vi "VIH UI - Append Control Rules - Ask If Add Duplicates.vi"(10 "Ctrl Rules (new)":T1[](array[typedef]), 11 "Ctrl Rules (existing)":T1[](array[typedef])) -> (2 "Ctrl Rules (new) out":T1[](array[typedef]))   [LabVIEW 2014]
doc: "::: VI Helpeks :::\nCopyright (c) 2000-2026 Konstantin Shifershteyn. All rights reserved."
uses:
  _VIH HelpGen.llb/VIH HelpGen Typedef - Cluster - Control Rule.ctl
  _VIH HelpGen.llb/VIH HelpGen Typedef - Enum - Description Mode.ctl
  _VIH HelpGen.llb/VIH HelpGen Typedef - Enum - Default,Enable,Disable.ctl
  _VIH HelpGen.llb/VIH HelpGen Typedef - Cluster - Enum Value Info.ctl
panel:
  # "VI Helpeks\nCopyright (c) 2012-2026 Konstantin Shifershteyn"
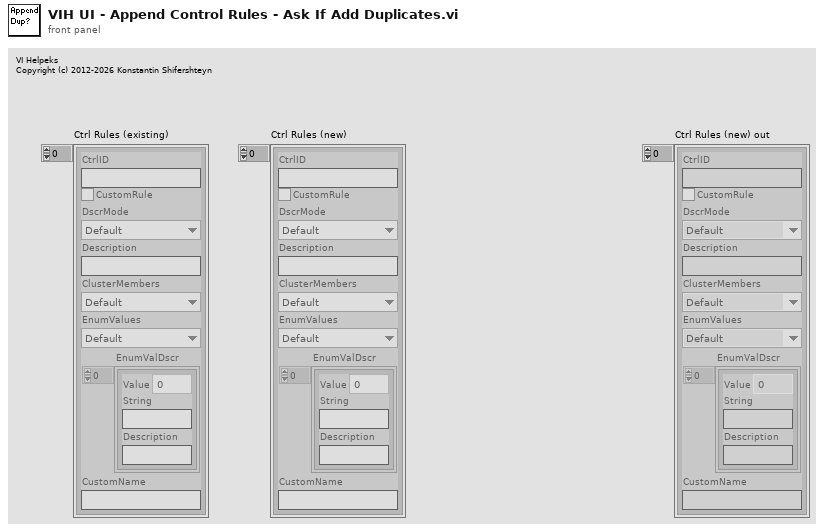
[diagram p1: front panel]
types:
  T1 = typedef "VIH HelpGen Typedef - Cluster - Control Rule.ctl" = cluster{"CtrlID":string, "CustomRule":bool, "DscrMode":T2, "Description":string, "ClusterMembers":T3, "EnumValues":T3, "EnumValDscr":T4[], "CustomName":string}
  T2 = typedef "VIH HelpGen Typedef - Enum - Description Mode.ctl" = enum16{"Default", "Description", "Description1", "Description2", "Custom", "None"}
  T3 = typedef "VIH HelpGen Typedef - Enum - Default,Enable,Disable.ctl" = enum16{"Default", "Enable", "Disable"}
  T4 = typedef "VIH HelpGen Typedef - Cluster - Enum Value Info.ctl" = cluster{"Value":ext, "String":string, "Description":string}
  T5 = enum16{"Left Button", "Center Button", "Right Button", "Window Close"}
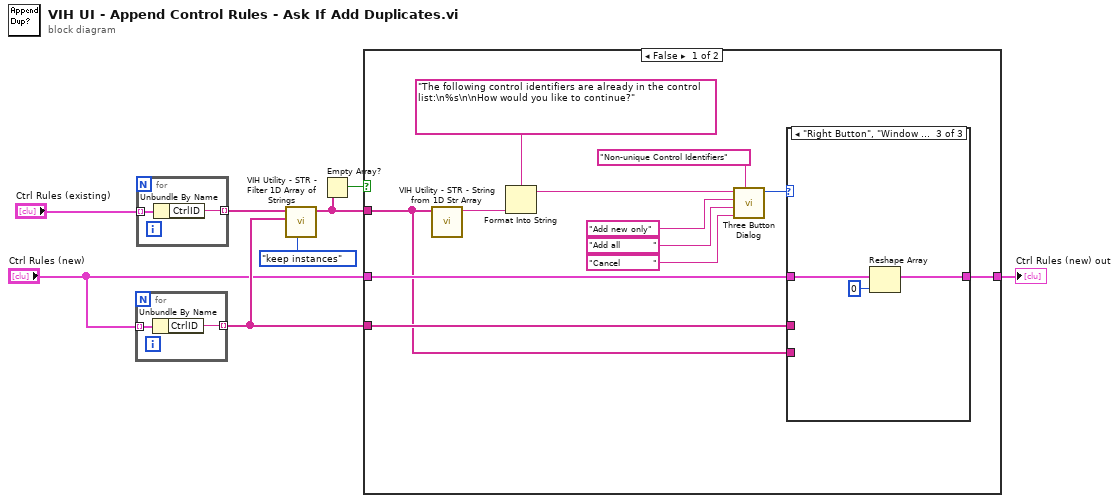
[diagram p0: block diagram]
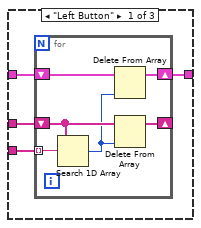
[diagram p2: hidden frame]
diagram:
  n1 = for {
    tunnel: "Ctrl Rules (new)" -> [w10] mode=indexing
    tunnel: [w9] -> w3 mode=indexing
    n2 = Unbundle By Name(w10) -> ("CtrlID"=w9:string)
  }
  n3 = for {
    tunnel: "Ctrl Rules (existing)" -> [w12] mode=indexing
    tunnel: [w11] -> w7 mode=indexing
    n4 = Unbundle By Name(w12) -> ("CtrlID"=w11:string)
  }
  n5 = call "VIH Utility - STR - Filter 1D Array of Strings.vi"("Action (keep instances)"=enum16{"keep instances", "remove instances"}."keep instances", "instances"=w3, "Array in"=w7) -> ("Array out"=w4:string[])  [unwired: 7 in, 1 out]
  n6 = Empty Array?(array=w4) -> (empty?=w5:bool)
  n7 = case shown="False" w5 {
    tunnel: w4 -> [w21 _]
    tunnel: w3 -> [w24 _]
    tunnel: "Ctrl Rules (new)" -> [w23 w39]
    tunnel: [w22 w39] -> w1
    frame False {
      n8 = call "VIH Utility - STR - String from 1D Str Array.vi"("Array in"=w21) -> ("String out"=w20:string)  [unwired: 6 in]
      n9 = Format Into String(format string="The following control identifiers are already in the control list:\n%s\n\nHow would you like to continue?", w20) -> (resulting string=w18:string)  [unwired: 2 in, 1 out]
      n10 = call <vilib>:"Three Button Dialog.vi"("Window Title (\"\")"="Non-unique Control Identifiers" ("Window Title (\"\")"), "Right Button Text (\"Cancel\")"="Cancel           " ("Right Button Text (\"Cancel\")"), "Center Button Text (\"No\")"="Add all           ", "Left Button Text (\"Yes\")"="Add new only" ("T button name (\"OK\")"), "message"=w18) -> ("Which Button?"=w19:T5)  [unwired: 6 in]
      n11 = case shown="\"Right Button\", \"Window Close\"" w19 {
        tunnel: w24 -> [w28 _ _]
        tunnel: w23 -> [w27 w35 w38]
        tunnel: [w26 w35 w37] -> w22
        tunnel: w21 -> [w25 _ _]
        frame "Left Button" {
          n12 = for {
            tunnel: w25 -> [w34] mode=indexing
            shift-right: [w30] -> _
            shift-left: w28 -> [w31]
            shift-right: [w32] -> w26
            shift-left: w27 -> [w33]
            n13 = Search 1D Array(1D array=w31, element=w34) -> (index of element=w29:i32)  [unwired: 1 in]
            n14 = Delete From Array(array=w33, index=w29) -> (array with subset deleted=w32:T1[])  [unwired: 1 in, 1 out]
            n15 = Delete From Array(array=w31, index=w29) -> (array with subset deleted=w30:string[])  [unwired: 1 in, 1 out]
          }
        }
        frame "Center Button" {
        }
        frame "Right Button", "Window Close" {
          n16 = Reshape Array(w38, 0 ("dimension size")) -> (w37:T1[])
        }
      }
    }
    frame True {
    }
  }
  "Ctrl Rules (new) out" <- w1
